vi "Total Analysis_2020_0820.vi"() -> ()   [LabVIEW 2018]
panel:
  in  "SR_enter":bool
  out "pta":string
  out "path":path
  out "folder list 3":string[](array[string])
  out "folder list 2":string[](array[string])
  out "Sample Sequence array":string[](array[string])
  out "SC array":T1(array[cluster])
  out "Path":path
  out "SB array":T1(array[cluster])
  in  "Folder Tab":T2(tab)
  out "folder list":string[](array[string])
  in  "Set Condition":T3={"+/- Point"=2000, "Cut Region"=500, "BL Selection"=enum."Div Value Mode BL", "STD Selection"=enum."DivSTD Mode STD", "D Th std xn"=1.0, "U Th std xn"=6.0, "MAX D time (ms)"=10.0, "LL BR (n)"=0, "LL BR T length (ms)"=0.0, "LL Retention (ms)"=0.0, "Read Region Point"=10000, "Filter Selection"=enum."Smooth", "STD smooth Point"=10, "MAX E_S time (ms)"=10.0}
  in  "S New Info and MiN out":T4={"Sample Sequence"="", "Right Read MIN"=6, "Filter P"=0, "STD Type"=enum."Region", "Base Table"=[], "Selection"=enum."10kHz", "noise MAX"=3, "Sample name"=""} {"Base Table"."Value 3" format="%.2g"}
  out "Sample name array":string[](array[string])
  in  "Control Tab":enum32{"ANAL", "BNAL", "CNAL", "TXT"}(tab)
  out "Count Graph":cluster{i32[], "Count":dbl[]}[](graph)
  out "Array 3":cluster{string, bool}[](array[cluster])
  out "P_F":string
  out "BNAL Sample":string[](array[string])
  out "SC#":i32
  out "Numeric":i32
  out "FC Progress":dbl(slide) scale=0.0..100.0
  out "Sample name":string
  out "Sample Sequence":string
  out "Total NGraph":dbl[][](graph)
  out "Raw data Graph":dbl[](graph)
  in  "TXT type":enum16{"Latest Type", "Q type", "W Type"}(ring)
  in  "xn":dbl=1.0 format="%#_13g"
  in  "string":string="txt"
  out "Total Folder 2":i32
  out "Present File# 2":i32
  out "F Progress 2":dbl(slide) scale=0.0..100.0
  out "Present Folder# 2":i32
  out "Total File 2":i32
  out "FD Progress#2":dbl(slide) scale=0.0..100.0
  out "x = y?":bool
  out "Filename":string
  in  "Selection":T5(ring)
  out "Total Folder":i32
  out "FD Progress":dbl(slide) scale=0.0..100.0
  out "Present Folder#":i32
  out "Present File#":i32
  out "F Progress":dbl(slide) scale=0.0..100.0
  out "Total File":i32
  out "Filename List":string[](array[string])
  out "error out出力":errorcluster caption="エラー出力"
  in  "error in":errorcluster caption="エラー入力（エラーなし）"
  in  "delete":bool
  in  "Go":bool
  in  "enter":bool
  out "folder name":path
  # "\\\\Rackstation\\analysis\\Chirality_N2\\DAsp\\DAsp_100k_Sample\\DAsp_100k_Sample#0001 Z_20200818_1003 INAN#2Pex0n1_D-Asp-10uM_EXZSV#10_20200818_1230_SGM  D0.540nm B100vsI_22.76_EP1_100_EP2_-100_DV_SC37-2706-28-G343.tdms"
  # "\\\\Rackstation\\analysis\\Chirality_N2\\DAsp\\DAsp_100k_Sample\\DAsp_100k_Sample#0001 Z_20200818_1003 INAN#2Pex0n1_D-Asp-10uM_EXZSV#10_20200818_1230_SGM  D0.540nm B100vsI_22.76_EP1_100_EP2_-100_DV_SC37-2706-28-G343.tdms"
  # "\\\\Rackstation\\analysis\\Chirality_N2\\DAsp\\DAsp_100k_Sample\\DAsp_100k_Sample#0001 Z_20200818_1003 INAN#2Pex0n1_D-Asp-10uM_EXZSV#10_20200818_1230_SGM  D0.540nm B100vsI_22.76_EP1_100_EP2_-100_DV_SC37-2706-28-G343.tdms"
  # "\\\\Rackstation\\analysis\\Chirality_N2\\DAsp\\DAsp_100k_Sample\\DAsp_100k_Sample#0001 Z_20200818_1003 INAN#2Pex0n1_D-Asp-10uM_EXZSV#10_20200818_1230_SGM  D0.540nm B100vsI_22.76_EP1_100_EP2_-100_DV_SC37-2706-28-G343.tdms"
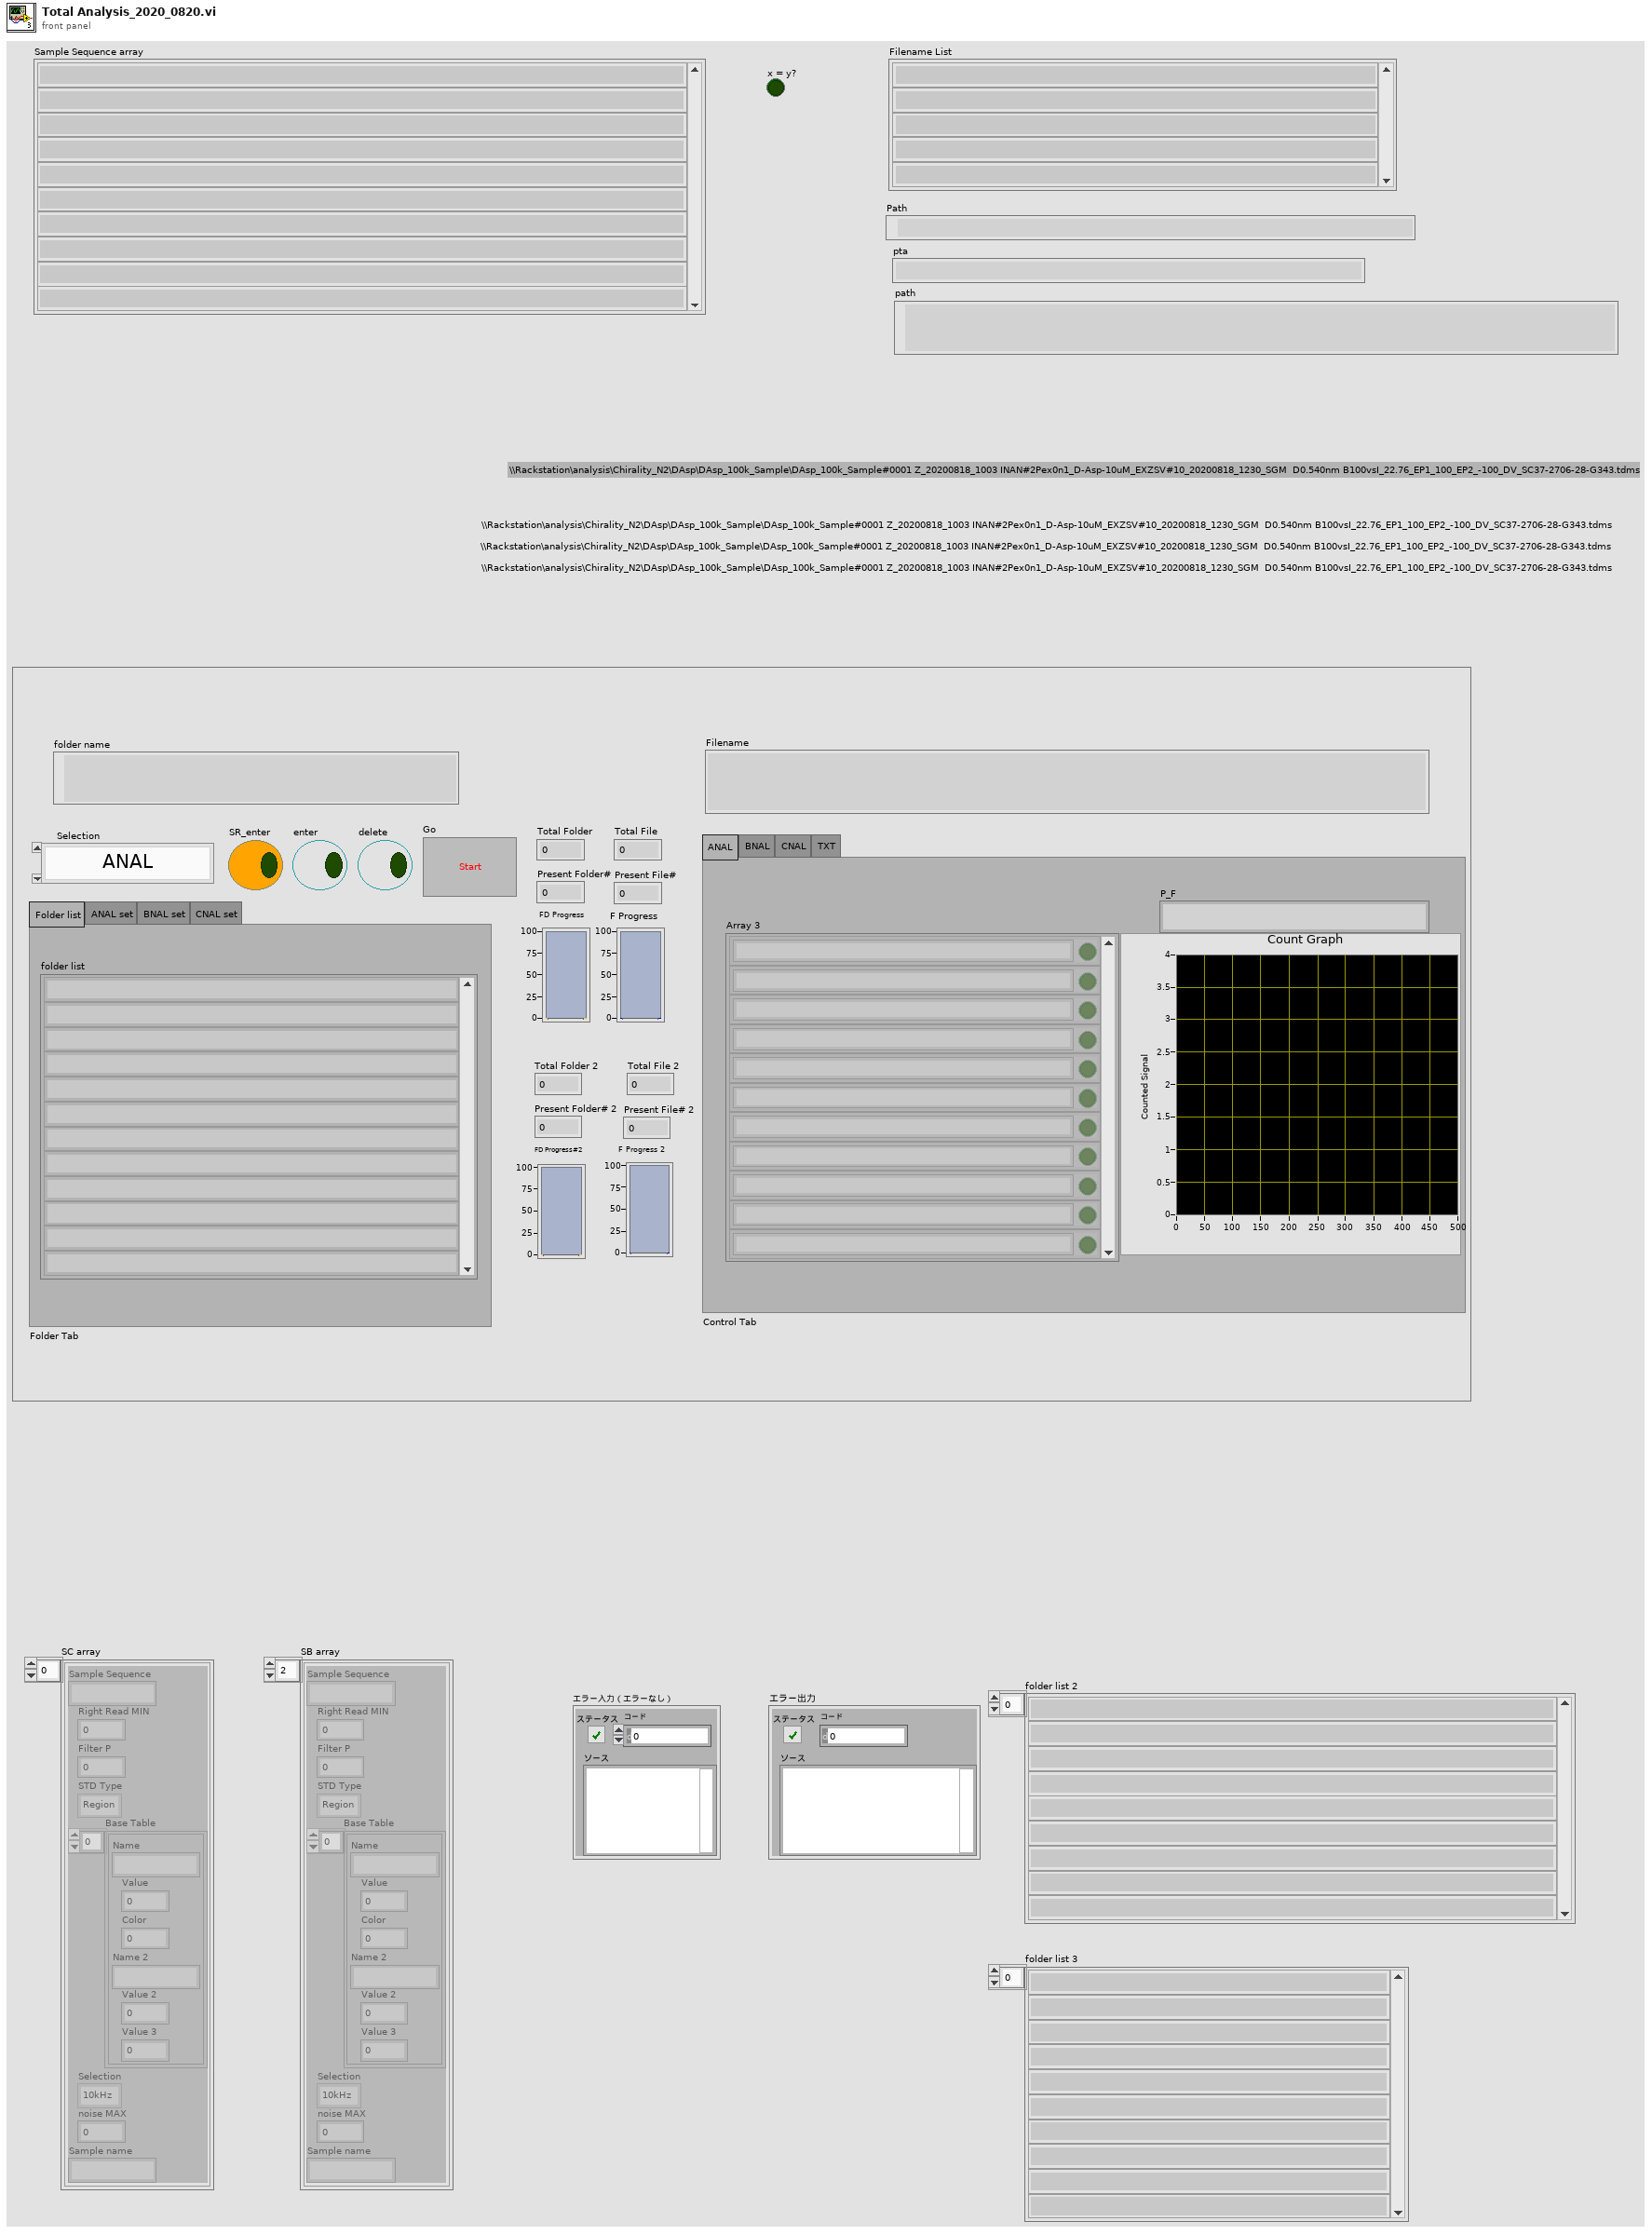
[diagram p1: front panel]
types:
  T1 = cluster{"Sample Sequence":string, "Right Read MIN":i32, "Filter P":i32, "STD Type":enum16{"Region", "Each", "Fixed"}, "Base Table":cluster{"Name":string, "Value":dbl, "Color":u32, "Name 2":string, "Value 2":dbl, "Value 3":dbl}[], "Selection":enum16{"10kHz", "100kHz"}, "noise MAX":i32, "Sample name":string}[]
  T2 = enum32{"Folder list", "ANAL set", "BNAL set", "CNAL set"}
  T3 = cluster{"+/- Point":i32, "Cut Region":i32, "BL Selection":enum16{"All Value Mode BL", "Div Value Mode BL", "Div Mean Mean BL", "Min Peak Value BL"}, "STD Selection":enum16{"All Value STD", "Div STD Mean STD", "DivSTD Mode STD"}, "D Th std xn":dbl, "U Th std xn":dbl, "MAX D time (ms)":dbl, "LL BR (n)":i32, "LL BR T length (ms)":dbl, "LL Retention (ms)":dbl, "Read Region Point":i32, "Filter Selection":enum16{"Mean", "Smooth"}, "STD smooth Point":i32, "MAX E_S time (ms)":dbl}
  T4 = cluster{"Sample Sequence":string, "Right Read MIN":i32, "Filter P":i32, "STD Type":enum16{"Region", "Each", "Fixed"}, "Base Table":cluster{"Name":string, "Value":dbl, "Color":u32, "Name 2":string, "Value 2":dbl, "Value 3":dbl}[], "Selection":enum16{"10kHz", "100kHz"}, "noise MAX":i32, "Sample name":string}
  T5 = enum16{"ANAL", "BNAL", "CNAL", "XNAL", "TXT to TDMS", "TANAL", "TDMS to TXT", "TABNAL"}
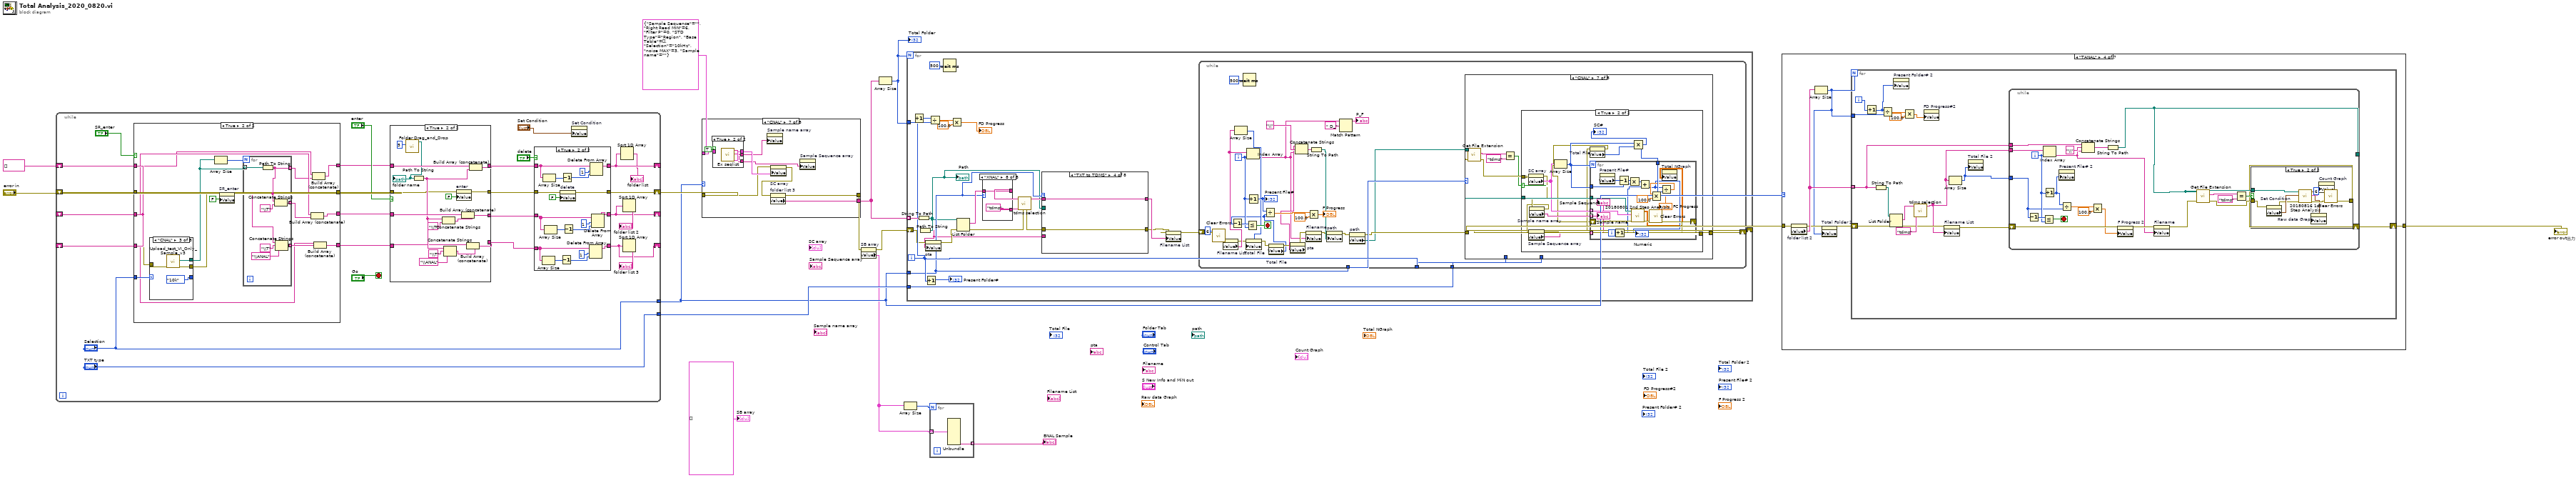
[diagram p0: block diagram]
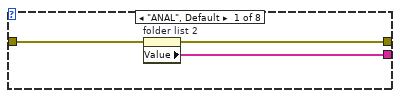
[diagram p2: hidden frame]
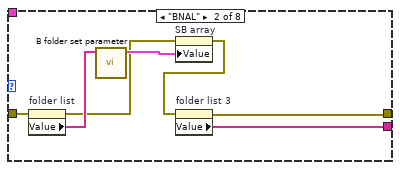
[diagram p3: hidden frame]
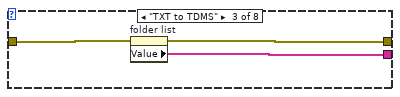
[diagram p4: hidden frame]
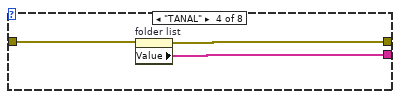
[diagram p5: hidden frame]
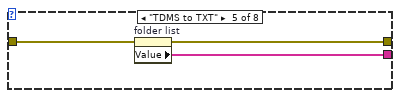
[diagram p6: hidden frame]
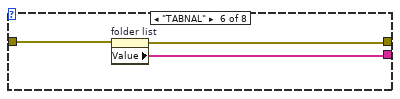
[diagram p7: hidden frame]
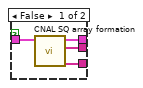
[diagram p8: hidden frame]
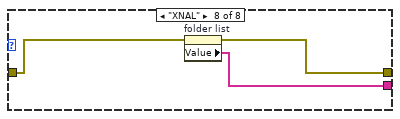
[diagram p9: hidden frame]
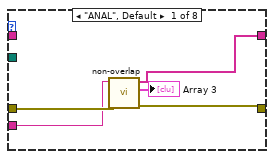
[diagram p17: hidden frame]
diagram:
  w8 = string[] []
  n1 = while {
    shift-right: [w38] -> _
    shift-left: w8 -> [w25]
    shift-right: [w33] -> w11
    shift-left: "error in" -> [w23]
    tunnel: ["Selection"] -> w10
    shift-right: [w35] -> _
    shift-left: w8 -> [w21]
    tunnel: ["TXT type"] -> w14
    shift-right: [w30] -> _
    shift-left: w8 -> [w19]
    stop <- "Go" stop-if-true
    n2 = case shown="True" "SR_enter" {
      tunnel: w23 -> [w46 w58]
      tunnel: [w46 w62] -> w22
      tunnel: [w45 w52] -> w24
      tunnel: w25 -> [w45 w50]
      tunnel: [w44 w54] -> w20
      tunnel: [w43 w49] -> w18
      tunnel: w21 -> [w44 w53]
      tunnel: w19 -> [w43 w47]
      tunnel: "Selection" -> [_ w59]
      frame False {
      }
      frame True {
        n3 = case shown="\"CNAL\"" w59 {
          tunnel: [enum16{"10k", "100k"}."10k" ("SHz_selection") enum16{"10k", "100k"}."10k" ("Hzselection") enum16{"10k", "100k"}."10k" ("Hzselection") enum16{"10k", "100k"}."10k" ("Hzselection") enum16{"10k", "100k"}."10k" ("Hzselection") enum16{"10k", "100k"}."100k" ("Hzselection") enum16{"10k", "100k"}."10k" ("Hzselection") w91] -> _
          tunnel: w58 -> [w64 w69 w73 w77 w81 w85 w89 w94]
          tunnel: [w63 w68 w72 w76 w80 w84 w88 w93] -> w57
          tunnel: [w65 w67 w71 w75 w79 w83 w87 w92] -> w56
          frame "ANAL", Default {
            n4 = call "Upload_test_VI _20230224.vi"("error in"=w64) -> ("error out"=w63:errorcluster, "selected F_array_Link"=w65:path[])  [unwired: 8 in, 1 out]
          }
          frame "BNAL" {
            n5 = call "Upload_test_VI_Only_Sample_v3.vi"("error in"=w69) -> ("error out"=w68:errorcluster, "S_Folder_path array"=w67:path[])  [unwired: 8 in, 1 out]
          }
          frame "CNAL" {
            n6 = call "Upload_test_VI_Only_Sample_v3.vi"("error in"=w73) -> ("error out"=w72:errorcluster, "S_Folder_path array"=w71:path[])  [unwired: 8 in, 1 out]
          }
          frame "TXT to TDMS" {
            n7 = call "Upload_test_VI.vi"("error in"=w77) -> ("error out"=w76:errorcluster, "selected F_array_Link"=w75:path[])  [unwired: 8 in, 1 out]
          }
          frame "TANAL" {
            n8 = call "Upload_test_VI.vi"("error in"=w81) -> ("error out"=w80:errorcluster, "selected F_array_Link"=w79:path[])  [unwired: 8 in, 1 out]
          }
          frame "TDMS to TXT" {
            n9 = call "Upload_test_VI.vi"("error in"=w85) -> ("error out"=w84:errorcluster, "selected F_array_Link"=w83:path[])  [unwired: 8 in, 1 out]
          }
          frame "TABNAL" {
            n10 = call "Upload_test_VI_Only_Sample_v3.vi"("error in"=w89) -> ("error out"=w88:errorcluster, "S_Folder_path array"=w87:path[])  [unwired: 8 in, 1 out]
          }
          frame "XNAL" {
            w91 = enum16{"10k", "100k"}."100k" ("SHz_selection")
            n11 = call "Upload_test_VI.vi"("error in"=w94, "SHz_selection"=w91) -> ("error out"=w93:errorcluster, "selected F_array_Link"=w92:path[])  [unwired: 7 in, 1 out]
          }
        }
        n12 = Array Size(array=w56) -> (size(s)=w60:i32)
        n13 = property on="SR_enter" class="Bool (strict)"(error in=w57, "Value"=FALSE ("10k_delete")) -> (error out=w62:errorcluster)  [unwired: 1 in, 1 out]
        n14 = for {
          N: w60 -> [_]
          tunnel: w56 -> [w101] mode=indexing
          tunnel: [w95] -> w51 mode=indexing
          tunnel: [w99] -> w55 mode=indexing
          tunnel: [w96] -> w48 mode=indexing
          n15 = Path To String(path=w101) -> (string=w95:string)
          n16 = Concatenate Strings(w95, "\\T" ("文字列")) -> (w99:string)
          n17 = Concatenate Strings(w95, "\\T" ("文字列"), "\\ANAL" ("文字列")) -> (w96:string)
        }
        n18 = Build Array (concatenate)(w53, w55) -> (w54:string[])
        n19 = Build Array (concatenate)(w50, w51) -> (w52:string[])
        n20 = Build Array (concatenate)(w47, w48) -> (w49:string[])
      }
    }
    n21 = case shown="True" "enter" {
      tunnel: w24 -> [w105 w122]
      tunnel: [w105 w121] -> w40
      tunnel: [w104 w120] -> w39
      tunnel: [w103 w117] -> w37
      tunnel: w20 -> [w103 w116]
      tunnel: [w102 w111] -> w32
      tunnel: w18 -> [w102 w110]
      tunnel: w22 -> [w104 w109]
      frame False {
      }
      frame True {
        n22 = call "Folder Drag_and_Drop.vi"("リング"=u16 5) -> ("Folder_Name"=w107:path)  [unwired: 10 in]
        "folder name" <- w107
        n23 = Path To String(path=w107) -> (string=w114:string)
        n24 = Concatenate Strings(w114, "\\T" ("文字列")) -> (w118:string)
        n25 = Concatenate Strings(w114, "\\T" ("文字列"), "\\ANAL" ("文字列")) -> (w112:string)
        n26 = property on="enter" class="Bool (strict)"(error in=w109, "Value"=FALSE ("ブール")) -> (error out=w120:errorcluster)  [unwired: 1 in, 1 out]
        n27 = Build Array (concatenate)(w116, w118) -> (w117:string[])
        n28 = Build Array (concatenate)(w110, w112) -> (w111:string[])
        n29 = Build Array (concatenate)(w122, w114) -> (w121:string[])
      }
    }
    n30 = case shown="True" "delete" {
      tunnel: w40 -> [w126 w141]
      tunnel: [w126 w143] -> w38
      tunnel: w39 -> [w125 w138]
      tunnel: [w125 w137] -> w33
      tunnel: [w124 w132] -> w35
      tunnel: w37 -> [w124 w133]
      tunnel: w32 -> [w123 w127]
      tunnel: [w123 w128] -> w30
      frame False {
      }
      frame True {
        n31 = Array Size(array=w127) -> (size(s)=w130:i32)
        n32 = Array Size(array=w141) -> (size(s)=w140:i32)
        n33 = Array Size(array=w133) -> (size(s)=w135:i32)
        n34 = property on="delete" class="Bool (strict)"(error in=w138, "Value"=FALSE ("削除")) -> (error out=w137:errorcluster)  [unwired: 1 in, 1 out]
        n35 = Decrement(x=w130) -> (x-1=w129:i32)
        n36 = Decrement(x=w140) -> (x-1=w139:i32)
        n37 = Decrement(x=w135) -> (x-1=w134:i32)
        n38 = Delete From Array(array=w127, length=1 ("長さ"), index=w129) -> (array with subset deleted=w128:string[])  [unwired: 1 out]
        n39 = Delete From Array(array=w141, length=1 ("長さ"), index=w139) -> (array with subset deleted=w143:string[])  [unwired: 1 out]
        n40 = Delete From Array(array=w133, length=1 ("長さ"), index=w134) -> (array with subset deleted=w132:string[])  [unwired: 1 out]
      }
    }
    n41 = property on="Set Condition" class="Clust (strict)"("Value"="Set Condition") -> ()  [unwired: 2 in, 2 out]
    n42 = Sort 1D Array(array=w38) -> (sorted array=→"folder list":string[])
    n43 = Sort 1D Array(array=w35) -> (sorted array=→"folder list 2":string[])
    n44 = Sort 1D Array(array=w30) -> (sorted array=→"folder list 3":string[])
  }
  n45 = case shown="\"CNAL\"" w10 {
    tunnel: w11 -> [w147 w149 w156 w159 w162 w165 w169 w183]
    tunnel: [w146 w153 w155 w158 w161 w164 w174 w182] -> w7
    tunnel: [w145 w152 w154 w157 w160 w163 w173 w184] -> w9
    tunnel: T4 {"Sample Sequence"="", "Right Read MIN"=6, "Filter P"=0, "STD Type"=enum."Region", "Base Table"=[], "Selection"=enum."10kHz", "noise MAX"=3, "Sample name"=""} ("S New Info and MiN out 2") -> [_ _ _ _ _ _ w172 _]
    frame "ANAL", Default {
      n46 = property on="folder list 2" class="Arr (strict)"(error in=w147) -> (error out=w146:errorcluster, "Value"=w145:string[])  [unwired: 1 in, 1 out]
    }
    frame "BNAL" {
      n47 = property on="folder list" class="Arr (strict)"(error in=w149) -> ("Value"=w151:string[])  [unwired: 1 in, 2 out]
      n48 = call "B folder set parameter.vi"("folder list"=w151) -> ("S array"=w150:T1)  [unwired: 10 in]
      n49 = property on="SB array" class="Arr (strict)"(error in=w149, "Value"=w150) -> (error out=w148:errorcluster)  [unwired: 1 in, 1 out]
      n50 = property on="folder list 3" class="Arr (strict)"(error in=w148) -> (error out=w153:errorcluster, "Value"=w152:string[])  [unwired: 1 in, 1 out]
    }
    frame "TXT to TDMS" {
      n51 = property on="folder list" class="Arr (strict)"(error in=w156) -> (error out=w155:errorcluster, "Value"=w154:string[])  [unwired: 1 in, 1 out]
    }
    frame "TANAL" {
      n52 = property on="folder list" class="Arr (strict)"(error in=w159) -> (error out=w158:errorcluster, "Value"=w157:string[])  [unwired: 1 in, 1 out]
    }
    frame "TDMS to TXT" {
      n53 = property on="folder list" class="Arr (strict)"(error in=w162) -> (error out=w161:errorcluster, "Value"=w160:string[])  [unwired: 1 in, 1 out]
    }
    frame "TABNAL" {
      n54 = property on="folder list" class="Arr (strict)"(error in=w165) -> (error out=w164:errorcluster, "Value"=w163:string[])  [unwired: 1 in, 1 out]
    }
    frame "CNAL" {
      n55 = case shown="True" TRUE {
        tunnel: w172 -> [w178 _]
        tunnel: [w177 w181] -> w171
        tunnel: [w176 w180] -> w168
        tunnel: [w175 w179] -> w167
        frame False {
          n56 = call "CNAL SQ array formation.vi"("S New Info and MiN out"=w178) -> ("Sample Sequence array"=w175:string[], "Sample name array"=w176:string[], "S array"=w177:T1)  [unwired: 8 in]
        }
        frame True {
          n57 = call "Ex seqlist.vi"() -> ("S array"=w181:T1, "selected Seq"=w179:string[], "selected sample name"=w180:string[])  [unwired: 9 in]
        }
      }
      n58 = property on="Sample name array" class="Arr (strict)"("Value"=w168) -> ()  [unwired: 2 in, 2 out]
      n59 = property on="SC array" class="Arr (strict)"(error in=w169, "Value"=w171) -> (error out=w170:errorcluster)  [unwired: 1 in, 1 out]
      n60 = property on="folder list 3" class="Arr (strict)"(error in=w170) -> (error out=w174:errorcluster, "Value"=w173:string[])  [unwired: 1 in, 1 out]
      n61 = property on="Sample Sequence array" class="Arr (strict)"("Value"=w167) -> ()  [unwired: 2 in, 2 out]
    }
    frame "XNAL" {
      n62 = property on="folder list" class="Arr (strict)"(error in=w183) -> (error out=w182:errorcluster, "Value"=w184:string[])  [unwired: 1 in, 1 out]
    }
  }
  n63 = property on="SB array" class="Arr (strict)"(error in=w7) -> (error out=w6:errorcluster, "Value"=w3:T1)  [unwired: 1 in, 1 out]
  n64 = Array Size(array=w9) -> (size(s)=w15:i32)
  "Total Folder" <- w15
  n65 = Array Size(array=w3) -> (size(s)=w5:i32)
  n66 = for {
    N: w15 -> [_]
    tunnel: w9 -> [w209] mode=indexing
    shift-right: [w208] -> w13
    shift-left: w6 -> [w193]
    tunnel: w15 -> [w205]
    tunnel: w10 -> [w191]
    tunnel: w14 -> [w201]
    i -> [w200]
    n67 = Increment(x=w200) -> (x+1=w203:i32)
    n68 = String To Path(string=w209) -> (path=w186:path)
    "Path" <- w186
    n69 = Path To String(path=w186) -> (string=w185:string)
    n70 = Increment(x=w200) -> (x+1=→"Present Folder#":i32)
    n71 = property on="pta" class="Str"(error in=w193, "Value"=w185) -> (error out=w192:errorcluster)  [unwired: 1 in, 1 out]
    n72 = Divide(x=w203, y=w205) -> (x/y=w207:dbl)
    n73 = Wait (ms)(milliseconds to wait=u32 500) -> ()  [unwired: 1 out]
    n74 = Multiply(x=w207, y=100.0) -> (x*y=→"FD Progress":dbl)
    n75 = List Folder(path=w186, error in=w192) -> (filenames=w199:string[], error out=w194:errorcluster)  [unwired: 2 in, 2 out]
    n76 = case shown="\"XNAL\"" w191 {
      tunnel: w199 -> [w231 w234 w236 w237 w240 w242 w244 w246]
      tunnel: [w231 w234 w236 w237 w240 w242 w244 w246] -> w198
      tunnel: ["tdms" ("string") "tdms" ("string") "string" "txt" ("string") "tdms" ("string") "txt" ("string") "tdms" ("string") "tdms" ("string")] -> w197
      frame "ANAL", Default {
      }
      frame "BNAL" {
      }
      frame "TXT to TDMS" {
      }
      frame "TANAL" {
      }
      frame "TDMS to TXT" {
      }
      frame "TABNAL" {
      }
      frame "CNAL" {
      }
      frame "XNAL" {
      }
    }
    n77 = call "tdms selection.vi"("error in"=w194, "string"=w197, "Filename List"=w198) -> ("Array 2"=w190:string[], "error out"=w188:errorcluster)  [unwired: 6 in, 1 out]
    n78 = case shown="\"TXT to TDMS\"" w191 {
      tunnel: w190 -> [_ w216 w218 w220 w222 w224 w226 _]
      tunnel: [w212 w216 w218 w220 w222 w224 w226 w227] -> w189
      tunnel: w188 -> [w214 w215 w217 w219 w221 w223 w225 w230]
      tunnel: [w213 w215 w217 w219 w221 w223 w225 w228] -> w187
      tunnel: w186 -> [_ _ _ _ _ _ _ _]
      tunnel: w185 -> [w211 _ _ _ _ _ _ w229]
      frame "ANAL", Default {
        n79 = call "non-overlap.vi"("error in"=w214, "String"=w211) -> ("error out"=w213:errorcluster, "Array 3"=→"Array 3":cluster{string, bool}[], "non-overlapped array"=w212:string[])  [unwired: 7 in]
      }
      frame "BNAL" {
      }
      frame "CNAL" {
      }
      frame "TXT to TDMS" {
      }
      frame "TANAL" {
      }
      frame "TDMS to TXT" {
      }
      frame "TABNAL" {
      }
      frame "XNAL" {
        n80 = call "non-overlap.vi"("error in"=w230, "String"=w229) -> ("error out"=w228:errorcluster, "non-overlapped array"=w227:string[])  [unwired: 7 in, 1 out]
      }
    }
    n81 = property on="Filename List" class="Arr (strict)"(error in=w187, "Value"=w189) -> (error out=w196:errorcluster)  [unwired: 1 in, 1 out]
    n82 = while {
      shift-right: [w270] -> w208
      shift-left: w196 -> [w260]
      tunnel: w191 -> [w269]
      tunnel: w201 -> [w268]
      tunnel: w200 -> [w267]
      i -> [w275]
      stop <- w274 stop-if-true
      n83 = call <vilib>:"Clear Errors.vi"("error in (no error)"=w260, "specific error code to clear (0: all)"=6) -> ("error out"=w251:errorcluster)  [unwired: 4 in, 1 out]
      n84 = property on="Filename List" class="Arr (strict)"(error in=w251) -> (error out=w256:errorcluster, "Value"=w257:string[])  [unwired: 1 in, 1 out]
      n85 = Array Size(array=w257) -> (size(s)=w255:i32)
      n86 = Wait (ms)(milliseconds to wait=u32 500) -> ()  [unwired: 1 out]
      n87 = property on="Total File" class="DigNum (strict)"(error in=w256, "Value"=w255) -> (error out=w254:errorcluster)  [unwired: 1 in, 1 out]
      n88 = Index Array(array=w257, index=w275) -> (element=w249:string)
      n89 = Increment(x=w275) -> (x+1=w277:i32)
      "Present File#" <- w277
      n90 = property on="Total File" class="DigNum (strict)"(error in=w254) -> (error out=w253:errorcluster, "Value"=w252:i32)  [unwired: 1 in, 1 out]
      n91 = Decrement(x=w252) -> (x-1=w278:i32)
      n92 = Less Or Equal?(x=w278, y=w275) -> (x <= y?=w274:bool)
      n93 = Divide(x=w277, y=w252) -> (x/y=w276:dbl)
      n94 = property on="pta" class="Str"(error in=w253) -> (error out=w259:errorcluster, "Value"=w258:string)  [unwired: 1 in, 1 out]
      n95 = Concatenate Strings(w258, "\\" ("文字列"), w249) -> (w279:string)
      n96 = property on="Filename" class="Str"(error in=w259, "Value"=w249) -> (error out=w264:errorcluster)  [unwired: 1 in, 1 out]
      n97 = Multiply(x=w276, y=100.0) -> (x*y=→"F Progress":dbl)
      n98 = String To Path(string=w279) -> (path=w265:path)
      n99 = property on="path" class="Path"(error in=w264, "Value"=w265) -> (error out=w263:errorcluster)  [unwired: 1 in, 1 out]
      n100 = Match Pattern(string=w249, regular expression=" D_") -> (before substring=→"P_F":string)  [unwired: 1 in, 3 out]
      n101 = property on="path" class="Path"(error in=w263) -> (error out=w262:errorcluster, "Value"=w261:path)  [unwired: 1 in, 1 out]
      n102 = case shown="\"CNAL\"" w269 {
        tunnel: w261 -> [_ w304 w323 w340 w352 w357 w359 _]
        tunnel: w262 -> [w284 w303 w322 w339 w351 w356 w362 w399]
        tunnel: [w285 w305 w318 w343 w348 w353 w358 w398] -> w270
        tunnel: w268 -> [_ _ w320 _ _ _ _ _]
        tunnel: w267 -> [_ w300 _ _ _ _ _ _]
        frame "ANAL", Default {
          n103 = property on="Filename List" class="Arr (strict)"(error in=w284) -> (error out=w280:errorcluster, "Value"=w283:string[])  [unwired: 1 in, 1 out]
          n104 = Array Size(array=w283) -> (size(s)=w282:i32)
          n105 = Equal To 0?(x=w282) -> (x = 0?=w281:bool)
          n106 = case shown="False" w281 {
            tunnel: [w287 w296] -> w285
            tunnel: w280 -> [w286 w296]
            frame False {
              n107 = property on="path" class="Path"(error in=w286) -> (error out=w289:errorcluster, "Value"=w290:path)  [unwired: 1 in, 1 out]
              n108 = property on="Set Condition" class="Clust (strict)"(error in=w289) -> (error out=w295:errorcluster, "Value"=w294:T3)  [unwired: 1 in, 1 out]
              n109 = call "20180816 1st Step Analysis.vi"("error in"=w295, "Set Condition"=w294, "F_name"=w290) -> ("error out"=w292:errorcluster, "Count Graph"=w293:cluster{i32[], "Count":dbl[]}[], "Raw data Graph"=w291:waveform(dbl))  [unwired: 6 in]
              n110 = property on="Count Graph" class="XYGraph (strict)"(error in=w292, "Value"=w293) -> (error out=w288:errorcluster)  [unwired: 1 in, 1 out]
              n111 = property on="Raw data Graph" class="WFGraph (strict)"(error in=w288, "Value"=w291) -> (error out=w287:errorcluster)  [unwired: 1 in, 1 out]
            }
            frame True {
            }
          }
        }
        frame "BNAL" {
          n112 = property on="SB array" class="Arr (strict)"(error in=w303) -> (error out=w302:errorcluster, "Value"=w301:T1)  [unwired: 1 in, 1 out]
          n113 = call <vilib>:"Get File Extension.vi"("error in (no error)"=w302, "file"=w304) -> ("error out"=w298:errorcluster, "lowercase file extension"=w308:string)  [unwired: 5 in, 3 out]
          n114 = Index Array(array=w301, index=w300) -> (element=w299:T4)
          n115 = property on="S New Info and MiN out" class="Clust (strict)"(error in=w298, "Value"=w299) -> (error out=w297:errorcluster)  [unwired: 1 in, 1 out]
          n116 = Equal?(x=w308, y="tdms") -> (x = y?=w306:bool)
          n117 = case shown="True" w306 {
            tunnel: [w309 w313] -> w305
            tunnel: w304 -> [_ w315]
            tunnel: w297 -> [w309 w317]
            frame False {
            }
            frame True {
              n118 = property on="S New Info and MiN out" class="Clust (strict)"(error in=w317) -> (error out=w316:errorcluster, "Value"=w314:T4)  [unwired: 1 in, 1 out]
              n119 = call "20180801 2nd Step Analysis.vi"("error in"=w316, "S New Info and MiN"=w314, "Filename"=w315) -> ("error out"=w311:errorcluster, "Raw data Graph"=w310:dbl[], "Total NGraph_MS"=w312:dbl[][])  [unwired: 6 in]
              n120 = property on="Total NGraph" class="IntGraph (strict)"("Value"=w312) -> ()  [unwired: 2 in, 2 out]
              n121 = property on="Raw data Graph" class="WFGraph (strict)"("Value"=w310) -> ()  [unwired: 2 in, 2 out]
              n122 = call <vilib>:"Clear Errors.vi"("error in (no error)"=w311) -> ("error out"=w313:errorcluster)  [unwired: 5 in, 1 out]
            }
          }
        }
        frame "TXT to TDMS" {
          n123 = case shown="\"Q type\", Default" w320 {
            tunnel: w323 -> [w326 w332 w334]
            tunnel: w322 -> [w328 w331 w336]
            tunnel: [w327 w330 w335] -> w321
            tunnel: [w325 w329 w333] -> w319
            frame "Q type", Default {
              n124 = call "TXT to TDMS Q.vi"("error in"=w328, "数値"="xn", "Original File name (TXT)"=w326) -> ("error out"=w327:errorcluster, "Raw data Graph"=w325:dbl[])  [unwired: 7 in]
            }
            frame "Latest Type" {
              n125 = call "TXT to TDMS.vi"("error in"=w331, "Original File name (TXT)"=w332) -> ("error out"=w330:errorcluster, "Raw data Graph"=w329:dbl[])  [unwired: 8 in]
            }
            frame "W Type" {
              n126 = call "TXT to TDMS W.vi"("error in"=w336, "Original File name (TXT)"=w334) -> ("error out"=w335:errorcluster, "Raw data Graph"=w333:dbl[])  [unwired: 8 in]
            }
          }
          n127 = property on="Raw data Graph" class="WFGraph (strict)"("Value"=w319) -> ()  [unwired: 2 in, 2 out]
          n128 = call <vilib>:"Clear Errors.vi"("error in (no error)"=w321) -> ("error out"=w318:errorcluster)  [unwired: 5 in, 1 out]
        }
        frame "TDMS to TXT" {
          n129 = call <vilib>:"Get File Extension.vi"("error in (no error)"=w339, "file"=w340) -> ("error out"=w338:errorcluster, "lowercase file extension"=w342:string)  [unwired: 5 in, 3 out]
          n130 = Equal?(x=w342, y="tdms") -> (x = y?=w337:bool)
          "x = y?" <- w337
          n131 = case shown="True" w337 {
            tunnel: [w344 w347] -> w343
            tunnel: w340 -> [_ w346]
            tunnel: w338 -> [w344 w345]
            frame False {
            }
            frame True {
              n132 = call "TDMS to TXT Modification.vi"("error in"=w345, "Original File name (TDMS)"=w346) -> ("error out"=w347:errorcluster)  [unwired: 8 in, 1 out]
            }
          }
        }
        frame "TANAL" {
          n133 = call "TXT to TDMS.vi"("error in"=w351, "Original File name (TXT)"=w352) -> ("error out"=w349:errorcluster, "Raw data Graph"=w350:dbl[])  [unwired: 8 in]
          n134 = property on="Raw data Graph" class="WFGraph (strict)"(error in=w349, "Value"=w350) -> (error out=w348:errorcluster)  [unwired: 1 in, 1 out]
        }
        frame "TABNAL" {
          n135 = call "TXT to TDMS.vi"("error in"=w356, "Original File name (TXT)"=w357) -> ("error out"=w354:errorcluster, "Raw data Graph"=w355:dbl[])  [unwired: 8 in]
          n136 = property on="Raw data Graph" class="WFGraph (strict)"(error in=w354, "Value"=w355) -> (error out=w353:errorcluster)  [unwired: 1 in, 1 out]
        }
        frame "CNAL" {
          n137 = call <vilib>:"Get File Extension.vi"("error in (no error)"=w362, "file"=w359) -> ("error out"=w361:errorcluster, "lowercase file extension"=w364:string)  [unwired: 5 in, 3 out]
          n138 = Equal?(x=w364, y="tdms") -> (x = y?=w360:bool)
          n139 = case shown="True" w360 {
            tunnel: [w365 w377] -> w358
            tunnel: w359 -> [_ w378]
            tunnel: w361 -> [w365 w376]
            frame False {
            }
            frame True {
              n140 = property on="SC array" class="Arr (strict)"(error in=w376) -> (error out=w369:errorcluster, "Value"=w375:T1)  [unwired: 1 in, 1 out]
              n141 = property on="Sample name array" class="Arr (strict)"(error in=w369) -> (error out=w368:errorcluster, "Value"=w372:string[])  [unwired: 1 in, 1 out]
              n142 = property on="Sample Sequence array" class="Arr (strict)"(error in=w368) -> (error out=w367:errorcluster, "Value"=w371:string[])  [unwired: 1 in, 1 out]
              n143 = Array Size(array=w375) -> (size(s)=w373:i32)
              n144 = property on="Total File" class="DigNum (strict)"(error in=w367) -> (error out=w366:errorcluster, "Value"=w374:i32)  [unwired: 1 in, 1 out]
              n145 = Multiply(x=w373, y=w374) -> (x*y=w370:i32)
              "SC#" <- w370
              n146 = for {
                N: w373 -> [_]
                tunnel: w378 -> [w397]
                tunnel: w375 -> [w393] mode=indexing
                shift-right: [w395] -> w377
                shift-left: w366 -> [w394]
                tunnel: w370 -> [w391]
                tunnel: w373 -> [w385]
                tunnel: w372 -> [w383] mode=indexing
                tunnel: w371 -> [w382] mode=indexing
                i -> [w392]
                n147 = property on="Present File#" class="DigNum (strict)"() -> ("Value"=w388:i32)  [unwired: 2 in, 2 out]
                n148 = Increment(x=w392) -> (x+1=w386:i32)
                n149 = Decrement(x=w388) -> (x-1=w384:i32)
                n150 = Multiply(x=w384, y=w385) -> (x*y=w387:i32)
                n151 = call "20180801 2nd Step Analysis.vi"("error in"=w394, "S New Info and MiN"=w393, "Filename"=w397) -> ("error out"=w396:errorcluster, "Total NGraph_MS"=w379:dbl[][])  [unwired: 6 in, 1 out]
                n152 = Add(x=w387, y=w386) -> (x+y=w380:i32)
                "Numeric" <- w380
                n153 = call <vilib>:"Clear Errors.vi"("error in (no error)"=w396) -> ("error out"=w395:errorcluster)  [unwired: 5 in, 1 out]
                n154 = Divide(x=w380, y=w391) -> (x/y=w381:dbl)
                n155 = Multiply(x=w381, y=100.0) -> (x*y=→"FC Progress":dbl)
                n156 = property on="Total NGraph" class="IntGraph (strict)"("Value"=w379) -> ()  [unwired: 2 in, 2 out]
                "Sample name" <- w383
                "Sample Sequence" <- w382
              }
            }
          }
        }
        frame "XNAL" {
          n157 = property on="Filename List" class="Arr (strict)"(error in=w399) -> (error out=w400:errorcluster, "Value"=w403:string[])  [unwired: 1 in, 1 out]
          n158 = Array Size(array=w403) -> (size(s)=w402:i32)
          n159 = Equal To 0?(x=w402) -> (x = 0?=w401:bool)
          n160 = case shown="False" w401 {
            tunnel: [w405 w411] -> w398
            tunnel: w400 -> [w410 w411]
            frame False {
              n161 = property on="path" class="Path"(error in=w410) -> (error out=w408:errorcluster, "Value"=w409:path)  [unwired: 1 in, 1 out]
              n162 = call "20220520 1st Step Analysis for 100kHz.vi"("error in"=w408, "F_name"=w409) -> ("error out"=w406:errorcluster, "Count Graph"=w407:cluster{i32[], "Count":dbl[]}[], "Raw data Graph"=w404:waveform(dbl))  [unwired: 6 in, 1 out]
              n163 = property on="Raw data Graph" class="WFGraph (strict)"("Value"=w404) -> ()  [unwired: 2 in, 2 out]
              n164 = property on="Count Graph" class="XYGraph (strict)"(error in=w406, "Value"=w407) -> (error out=w405:errorcluster)  [unwired: 1 in, 1 out]
            }
            frame True {
            }
          }
        }
      }
    }
  }
  n165 = for {
    N: w5 -> [_]
    tunnel: w3 -> [w413] mode=indexing
    tunnel: [w412] -> w4 mode=indexing
    n166 = Unbundle(w413) -> ("Sample name"=w412:string)  [unwired: 7 out]
  }
  "BNAL Sample" <- w4
  n167 = case shown="\"TANAL\"" w10 {
    tunnel: w13 -> [w414 w415 w416 w421 w468 w469 w470]
    tunnel: [w414 w415 w416 w418 w468 w469 w470] -> w12
    frame "ANAL", Default {
    }
    frame "BNAL" {
    }
    frame "TXT to TDMS" {
    }
    frame "TANAL" {
      n168 = property on="folder list 2" class="Arr (strict)"(error in=w421) -> (error out=w419:errorcluster, "Value"=w420:string[])  [unwired: 1 in, 1 out]
      n169 = Array Size(array=w420) -> (size(s)=w417:i32)
      n170 = property on="Total Folder 2" class="DigNum (strict)"("Value"=w417) -> ()  [unwired: 2 in, 2 out]
      n171 = for {
        N: w417 -> [_]
        tunnel: w417 -> [w435]
        tunnel: w420 -> [w432] mode=indexing
        shift-right: [w422] -> w418
        shift-left: w419 -> [w426]
        i -> [w433]
        n172 = Increment(x=w433) -> (x+1=w431:i32)
        n173 = String To Path(string=w432) -> (path=w434:path)
        n174 = Divide(x=w431, y=w435) -> (x/y=w437:dbl)
        n175 = List Folder(path=w434, error in=w426) -> (filenames=w428:string[], error out=w425:errorcluster)  [unwired: 2 in, 2 out]
        n176 = property on="Present Folder# 2" class="DigNum (strict)"("Value"=w431) -> ()  [unwired: 2 in, 2 out]
        n177 = Multiply(x=w437, y=100.0) -> (x*y=w429:dbl)
        n178 = call "tdms selection.vi"("string"="tdms", "Filename List"=w428) -> ("Array 2"=w423:string[])  [unwired: 7 in, 2 out]
        n179 = property on="FD Progress#2" class="Slide (strict)"("Value"=w429) -> ()  [unwired: 2 in, 2 out]
        n180 = property on="Filename List" class="Arr (strict)"(error in=w425, "Value"=w423) -> (error out=w424:errorcluster)  [unwired: 1 in, 1 out]
        n181 = Array Size(array=w423) -> (size(s)=w430:i32)
        n182 = property on="Total File 2" class="DigNum (strict)"("Value"=w430) -> ()  [unwired: 2 in, 2 out]
        n183 = while {
          tunnel: w432 -> [w454]
          tunnel: w423 -> [w453]
          tunnel: w430 -> [w451]
          shift-right: [w438] -> w422
          shift-left: w424 -> [w447]
          tunnel: [w446] -> _
          i -> [w452]
          stop <- w450 stop-if-true
          n184 = Decrement(x=w451) -> (x-1=w456:i32)
          n185 = Less Or Equal?(x=w456, y=w452) -> (x <= y?=w450:bool)
          n186 = Index Array(array=w453, index=w452) -> (element=w441:string)
          n187 = Increment(x=w452) -> (x+1=w439:i32)
          n188 = property on="Present File# 2" class="DigNum (strict)"("Value"=w439) -> ()  [unwired: 2 in, 2 out]
          n189 = Divide(x=w439, y=w451) -> (x/y=w455:dbl)
          n190 = Concatenate Strings(w454, "\\" ("文字列"), w441) -> (w457:string)
          n191 = Multiply(x=w455, y=100.0) -> (x*y=w440:dbl)
          n192 = String To Path(string=w457) -> (path=w446:path)
          n193 = property on="F Progress 2" class="Slide (strict)"("Value"=w440) -> ()  [unwired: 2 in, 2 out]
          n194 = property on="Filename" class="Str"("Value"=w441) -> ()  [unwired: 2 in, 2 out]
          n195 = call <vilib>:"Get File Extension.vi"("error in (no error)"=w447, "file"=w446) -> ("error out"=w443:errorcluster, "lowercase file extension"=w445:string)  [unwired: 5 in, 3 out]
          n196 = Equal?(x=w445, y="tdms") -> (x = y?=w442:bool)
          n197 = case shown="True" w442 {
            tunnel: [w458 w460] -> w438
            tunnel: w446 -> [_ w466]
            tunnel: w443 -> [w458 w464]
            frame False {
            }
            frame True {
              n198 = property on="Set Condition" class="Clust (strict)"(error in=w464) -> (error out=w463:errorcluster, "Value"=w465:T3)  [unwired: 1 in, 1 out]
              n199 = call "20180816 1st Step Analysis.vi"("error in"=w463, "Set Condition"=w465, "F_name"=w466) -> ("error out"=w467:errorcluster, "Count Graph"=w461:cluster{i32[], "Count":dbl[]}[], "Raw data Graph"=w462:waveform(dbl))  [unwired: 6 in]
              n200 = property on="Raw data Graph" class="WFGraph (strict)"("Value"=w462) -> ()  [unwired: 2 in, 2 out]
              n201 = property on="Count Graph" class="XYGraph (strict)"("Value"=w461) -> ()  [unwired: 2 in, 2 out]
              n202 = call <vilib>:"Clear Errors.vi"("error in (no error)"=w467, "specific error code to clear (0: all)"=6) -> ("error out"=w460:errorcluster)  [unwired: 4 in, 1 out]
            }
          }
        }
      }
    }
    frame "TDMS to TXT" {
    }
    frame "TABNAL" {
    }
    frame "CNAL" {
    }
  }
  "error out出力" <- w12
  "SB array" <- T1 [] ("S array")
